vi "Test App Broadcast Nested Process Messages.vi"(8 "error in (no error)":errorcluster, 11 "Application Test In":refnum<class "Application Dev Test.lvclass">) -> (0 "error out":errorcluster, 3 "Application Test Out":refnum<class "Application Dev Test.lvclass">)   [LabVIEW 2020, in "Application Dev Test.lvclass"]
uses:
  Application Dev Test.lvclass
  C:/Program Files (x86)/National Instruments/LabVIEW 2020/vi.lib/Astemes/LUnit/Test Case.lvclass
  source/Framework Test Suite/Mock Process/Mock Process.lvclass
  C:/git/astemes-triarc-framework/source/Framework/Process/Process.lvclass
  source/Framework/Application/Application.lvclass
  source/Framework/Process/Process.lvclass/Process.ctl
  <vilib>/Astemes/LUnit/Test Case.lvclass/Test Case.ctl
  c27f4279-7cb7-4f54-8dc5-63ff7bac36e5.vi
  76411ce1-69dc-435f-b6fb-e9cd8e6b3fac.vi
  source/Framework/Process/Private/SubVIs/Wait for finish.vi
  source/Framework/Process/Private/SubVIs/Set Lifecycle State.vi
  source/Framework/Process/Protected/Messaging/Send Message.vi
  source/Framework/Broadcast Event Dequeuers/Execution timer.vi
  <vilib>/Astemes/LUnit/Append Pass Result.vi
  <vilib>/Astemes/LUnit/Append Fail Result.vi
  c27f4279-7cb7-4f54-8dc5-63ff7bac36e5.vi/9c5d11cd-9439-4240-a1ee-d9baace9c924.vi
  76411ce1-69dc-435f-b6fb-e9cd8e6b3fac.vi/9c5d11cd-9439-4240-a1ee-d9baace9c924.vi
  source/Framework/Process/Private/SubVIs/Handle Debug Data.vi
  <vilib>/Astemes/LUnit/Run In UI.vi
  source/Framework/Logging/Log Debug.vi
  <vilib>/AdvancedString/1D String Array to Delimited String.vi
  <vilib>/Utility/High Resolution Relative Seconds.vi
  <vilib>/Utility/error.llb/Clear Errors.vi
  source/Framework/Process/Public/Lifecycle/Get Lifecycle State.vi
  <vilib>/Utility/error.llb/Error Cluster From Error Code.vi
  source/Framework/Process/Public/Read Name.vi
  source/Framework/Broadcast Event Dequeuers/Dequeue Broadcast Message.vi
  source/Framework/Callback/Callback.lvclass
  source/Framework/Process/Process.lvclass
  Application Dev Test.lvclass/Application Dev Test.ctl
  source/Framework/Broadcast Event Dequeuers/Broadcast Event Dequeuers.lvlib
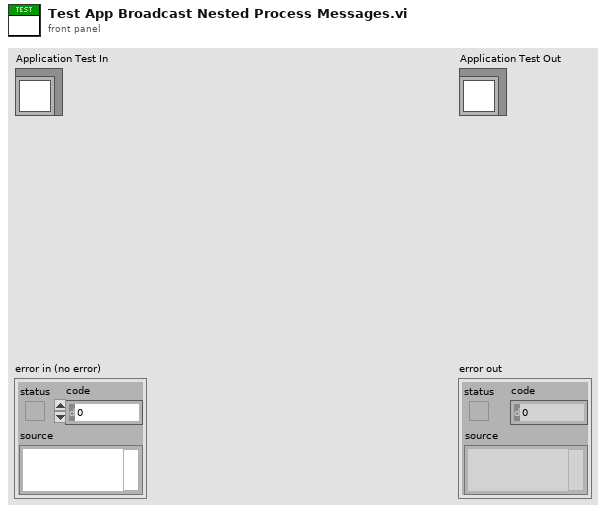
[diagram p1: front panel]
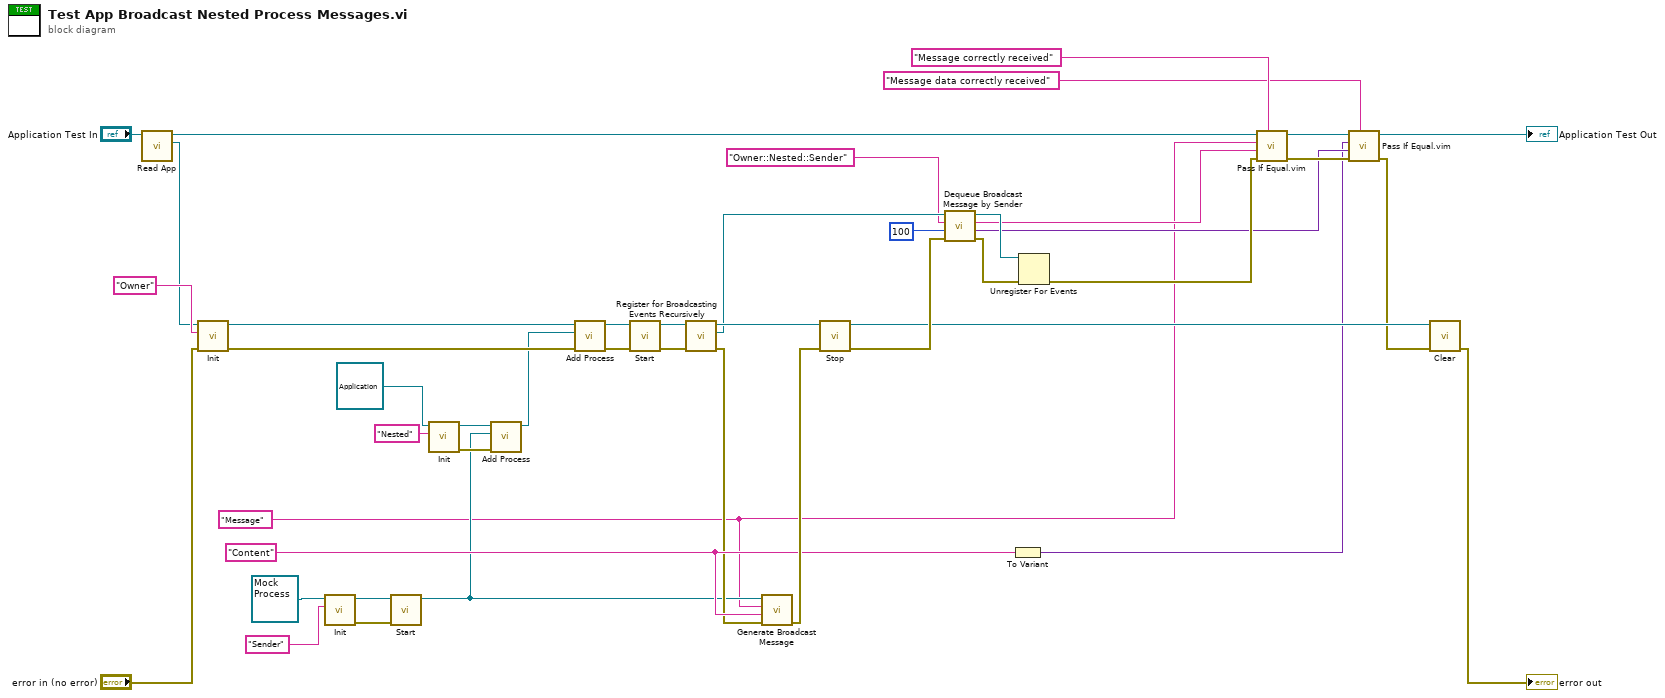
[diagram p0: block diagram]
diagram:
  w24 = "Content" ("Message")
  w2 = "Message" ("Message")
  n1 = call "Read App.vi"("Application Test In"="Application Test In") -> ("App out"=w27:refnum<class "Application.lvclass">, "Application Test Out"=w28:refnum<class "Application Dev Test.lvclass">)  [unwired: 8 in, 1 out]
  n2 = call-dynamic "Init.vi"("error in (no error)"="error in (no error)", "Name"="Owner" ("Message"), "Process In"=w27) -> ("error out"=w43:errorcluster, "Process Out"=w44:refnum<class "Application.lvclass">)  [unwired: 7 in]
  n3 = call-dynamic "Init.vi"("Name"="Sender" ("Message"), "Mock Process In"=refnum<class "Mock Process.lvclass"> refnum ("Mock Process.lvclass")) -> ("error out"=w31:errorcluster, "Mock Process Out"=w30:refnum<class "Mock Process.lvclass">)  [unwired: 8 in]
  n4 = call "Start.vi"("error in (no error)"=w31, "Process In"=w30) -> ("Process Out"=w9:refnum<class "Mock Process.lvclass">)  [unwired: 7 in, 2 out]
  n5 = call-dynamic "Init.vi"("Name"="Nested", "Process In"=refnum<class "Application.lvclass"> refnum ("Process Out")) -> ("error out"=w12:errorcluster, "Process Out"=w11:refnum<class "Application.lvclass">)  [unwired: 8 in]
  n6 = call "Add Process.vi"("error in (no error)"=w12, "Process"=w9, "Application In"=w11) -> ("Application Out"=w8:refnum<class "Application.lvclass">)  [unwired: 7 in, 1 out]
  n7 = call "Add Process.vi"("error in (no error)"=w43, "Process"=w8, "Application In"=w44) -> ("error out"=w19:errorcluster, "Application Out"=w4:refnum<class "Application.lvclass">)  [unwired: 7 in]
  n8 = call "Start.vi"("error in (no error)"=w19, "Process In"=w4) -> ("error out"=w5:errorcluster, "Process Out"=w3:refnum<class "Application.lvclass">)  [unwired: 7 in, 1 out]
  n9 = call "Register for Broadcasting Events Recursively.vi"("error in (no error)"=w5, "Application In"=w3) -> ("error out"=w17:errorcluster, "Event Registration Refnum Out"=w16:refnum<event-registration>, "Application Out"=w18:refnum<class "Application.lvclass">)  [unwired: 7 in]
  n10 = call "Generate Broadcast Message.vi"("error in (no error)"=w17, "Message Data"=w24, "Message"=w2, "Mock Process In"=w9) -> ("error out"=w26:errorcluster)  [unwired: 6 in, 1 out]
  n11 = call "Stop.vi"("error in (no error)"=w26, "Process In"=w18) -> ("error out"=w42:errorcluster, "Process Out"=w15:refnum<class "Application.lvclass">)  [unwired: 7 in, 1 out]
  n12 = call "Dequeue Broadcast Message by Sender.vi"("error in (no error)"=w42, "Timeout (-1)"=100, "Sender"="Owner::Nested::Sender" ("Message"), "Event Registration Refnum"=w16) -> ("error out"=w20:errorcluster, "Message Data"=w22:variant, "Message"=w23:string, "Event Registration Refnum Out"=w40:refnum<event-registration>)  [unwired: 3 in, 1 out]
  n13 = To Variant(anything=w24) -> (Variant=w1:variant)
  n14 = Unregister For Events(event registration refnum=w40, error in=w20) -> (error out=w36:errorcluster)
  n15 = call "Pass If Equal.vim"("Description"="Message correctly received", "error in (no error)"=w36, "Actual"=w23, "Expected"=w2, "LUnit Test Case In"=w28) -> ("error out"=w37:errorcluster, "LUnit Test Case Out"=w38:refnum<class "Application Dev Test.lvclass">)  [unwired: 5 in]
  n16 = call "Pass If Equal.vim"("Description"="Message data correctly received", "error in (no error)"=w37, "Actual"=w22, "Expected"=w1, "LUnit Test Case In"=w38) -> ("error out"=w14:errorcluster, "LUnit Test Case Out"=→"Application Test Out":refnum<class "Application Dev Test.lvclass">)  [unwired: 5 in]
  n17 = call-dynamic "Clear.vi"("error in (no error)"=w14, "Application In"=w15) -> ("error out"=→"error out":errorcluster)  [unwired: 9 in]
